vi "Acquire Data.vi"(7 "user event":T2, 8 "error in (no error)":errorcluster, 9 "UI Refs":T1, 10 "Waveforms":waveform(dbl)[](array[waveform]), 11 "Pressure Gain":refnum<class "Pressure Gain.lvclass">) -> (0 "error out":errorcluster, 3 "Pressure Gain out":refnum<class "Pressure Gain.lvclass">)   [LabVIEW 2025, in "Flow Grind.lvlib" / "Pressure Gain.lvclass"]
uses:
  Pressure Gain.lvclass
  Users/Public/Documents/Sandia National Labs/TSS Plugin/CEF.lvlibp/Node/UserEventRef.ctl
  Users/Public/Documents/Sandia National Labs/TSS Plugin/Tests/XY Plotter.lvlibp/XY  Plotter/XY Plotter.lvclass
  Users/Public/Documents/Sandia National Labs/TSS Plugin/CEF.lvlibp/Node/CEF_Node.lvclass
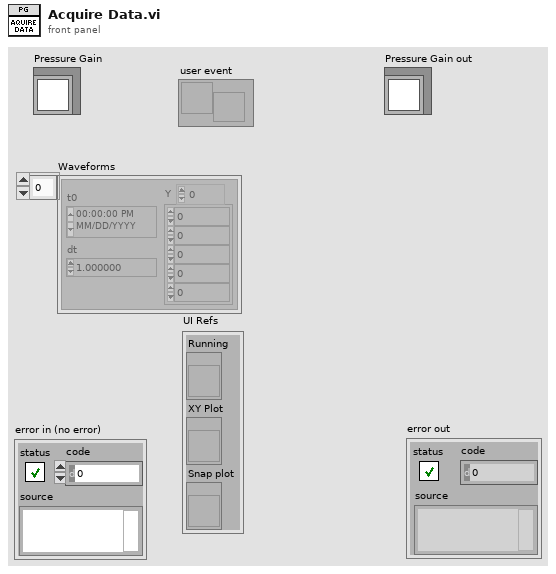
[diagram p1: front panel]
types:
  T1 = cluster{"Running":refnum<vi>, "XY Plot":refnum<vi>, "Snap plot":refnum<vi>}
  T2 = typedef "CEF.lvlibp/CEF_Node.lvclass/UserEventRef.ctl" = refnum<user-event>
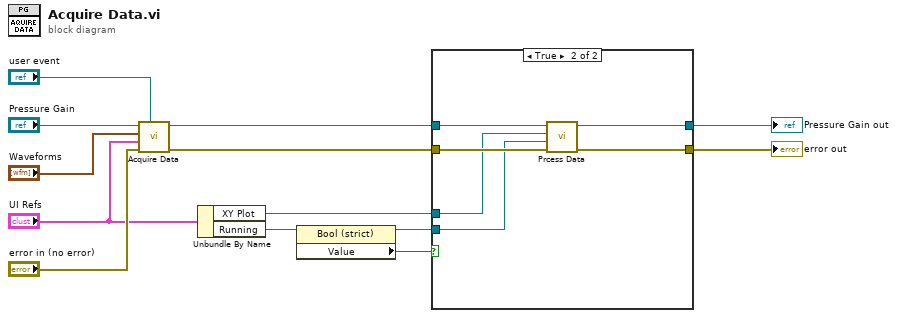
[diagram p0: block diagram]
diagram:
  n1 = call-parent "Acquire Data.vi"("user event"="user event", "error in (no error)"="error in (no error)", "UI Refs"="UI Refs", "Waveforms"="Waveforms", "XY Plotter"="Pressure Gain") -> ("error out"=w6:errorcluster, "XY Plotter out"=w5:refnum<class "Pressure Gain.lvclass">)  [unwired: 5 in]
  n2 = Unbundle By Name("UI Refs") -> ("XY Plot"=w2:refnum<vi>, "Running"=w9:refnum<vi>)
  n3 = property class="Bool (strict)"(reference=w9) -> (reference out=w1:refnum<vi>, "Value"=w7:bool)  [unwired: 1 in, 1 out]
  n4 = case shown="True" w7 {
    tunnel: w6 -> [w14 w19]
    tunnel: w5 -> [w15 w21]
    tunnel: [w15 w20] -> w4
    tunnel: [w14 w18] -> w3
    tunnel: w2 -> [_ w17]
    tunnel: w1 -> [_ w16]
    frame False {
    }
    frame True {
      n5 = call "Prcess Data.vi"("error in (no error)"=w19, "Running"=w16, "XY Plot"=w17, "PG"=w21) -> ("error out"=w18:errorcluster, "PG"=w20:refnum<class "Pressure Gain.lvclass">)  [unwired: 6 in]
    }
  }
  "error out" <- w3
  "Pressure Gain out" <- w4
